vi "Main2.vi"() -> ()   [LabVIEW 2024]
uses:
  Global 1.vi
  Control 1.ctl
panel:
  in  "Array 3":string[][](array[string])=[["dsfds", "-797", "-798", "-1.00", "No Alarm", "<", "12"]]
  out "Waveform Graph":dbl[][](graph)
  out "Array 2":string[][](array[string])
  out "# Of Curr Paramters":dbl
  out "# Of total Paramters":dbl
  in  "Print Button":bool
  out "Current Running Test":string
  in  "Rate of change":T1(array[cluster])
  out "Numeric":dbl
  out "error out":errorcluster
  out "Time Elapsed?":bool=TRUE
  out "Paused?":bool
  in  "error in (no error)":errorcluster
  in  "Select Time":enum16{"Reset", "Start", "Pause", "Unpause"}(ring)=enum."Start"
  in  "Array 4":T2(array[cluster])
  out "Table Control":string[][](table)
  # "Timer"
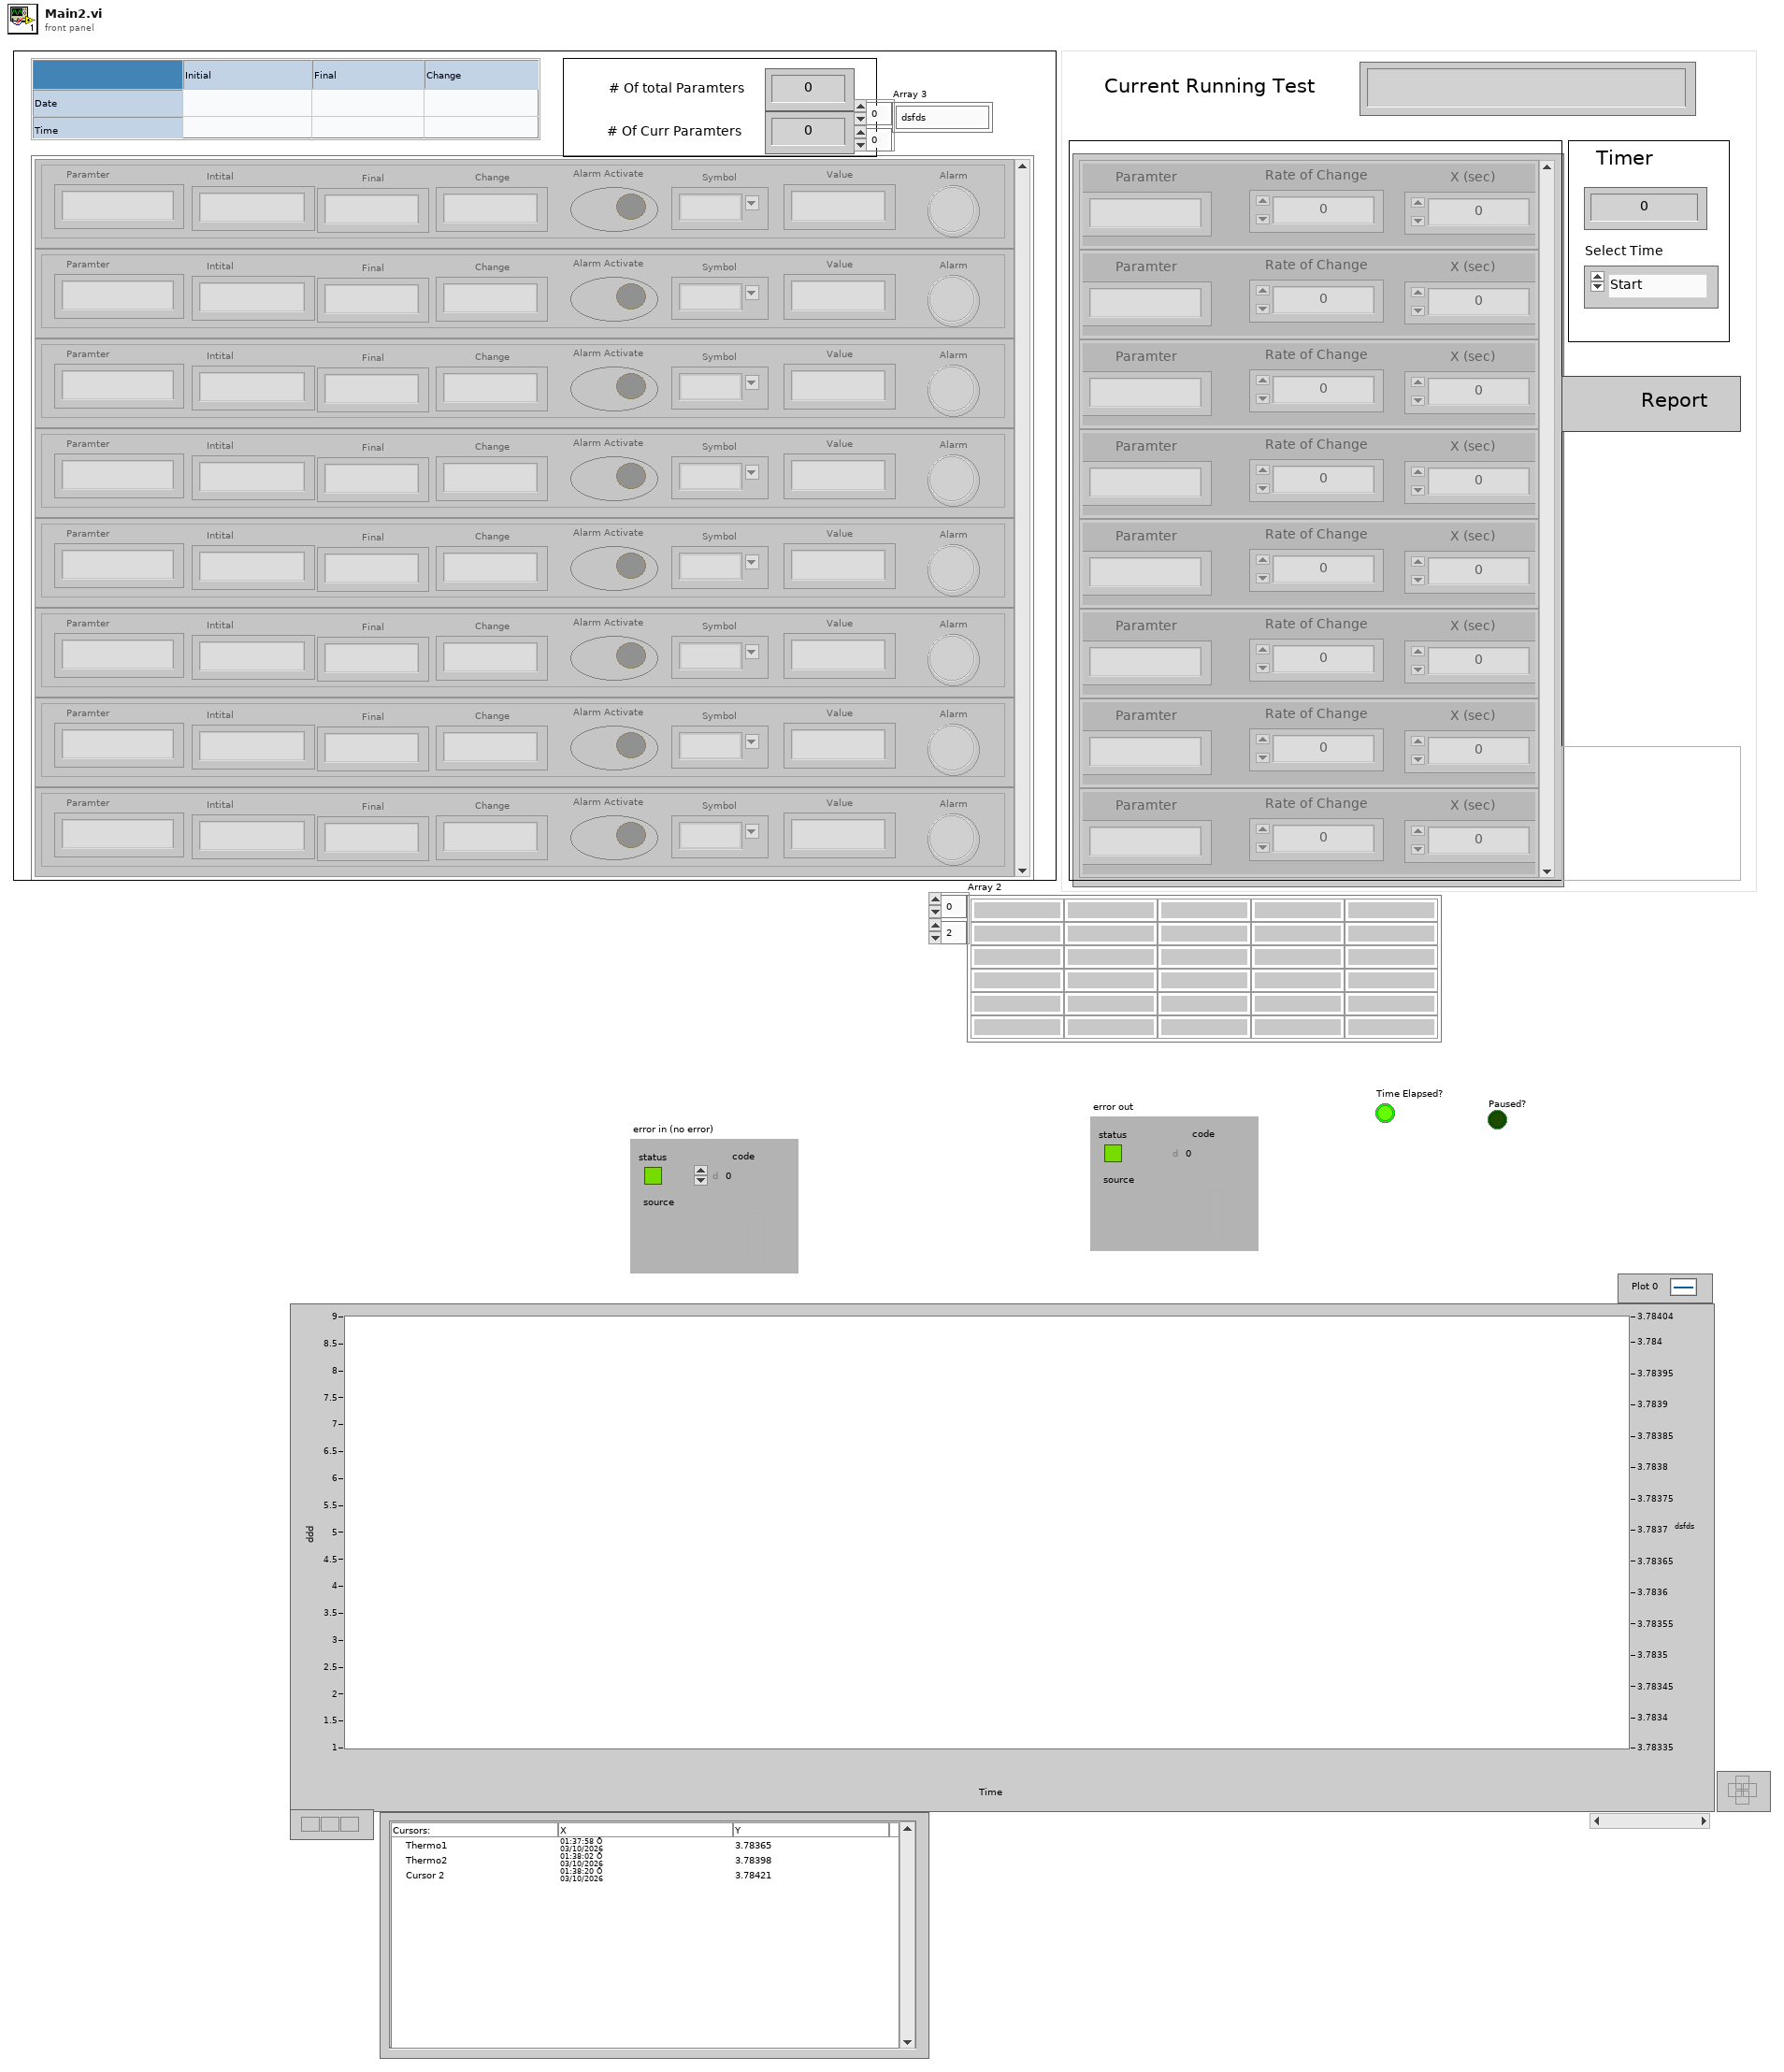
[diagram p1: front panel]
types:
  T1 = cluster{"Paramter":string, "Rate of Change":dbl, "X (sec)":dbl}[]
  T2 = cluster{"Paramter":string, "Intital ":string, "Final":string, "Change":string, "Alarm Activate ":bool, "Symbol":string, "Value":string, "Alarm":bool}[]
  T3 = cluster{"Paramter":string, "Rate of Change":dbl, "X (min)":dbl}[]
  T4 = cluster{"Paramter":string, "Rate of Change":dbl, "X Min":string}[]
  T5 = typedef "Control 1.ctl" = enum16{"Start", "Initialize"}
  T6 = cluster{"Paramter":string, "Rate of Change":dbl, "X (min)":dbl}
  T7 = cluster{"Paramter":string, "Intital ":string, "Final":string, "Change":string, "Alarm Activate ":bool, "Symbol":string, "Value":string, "Alarm":bool}
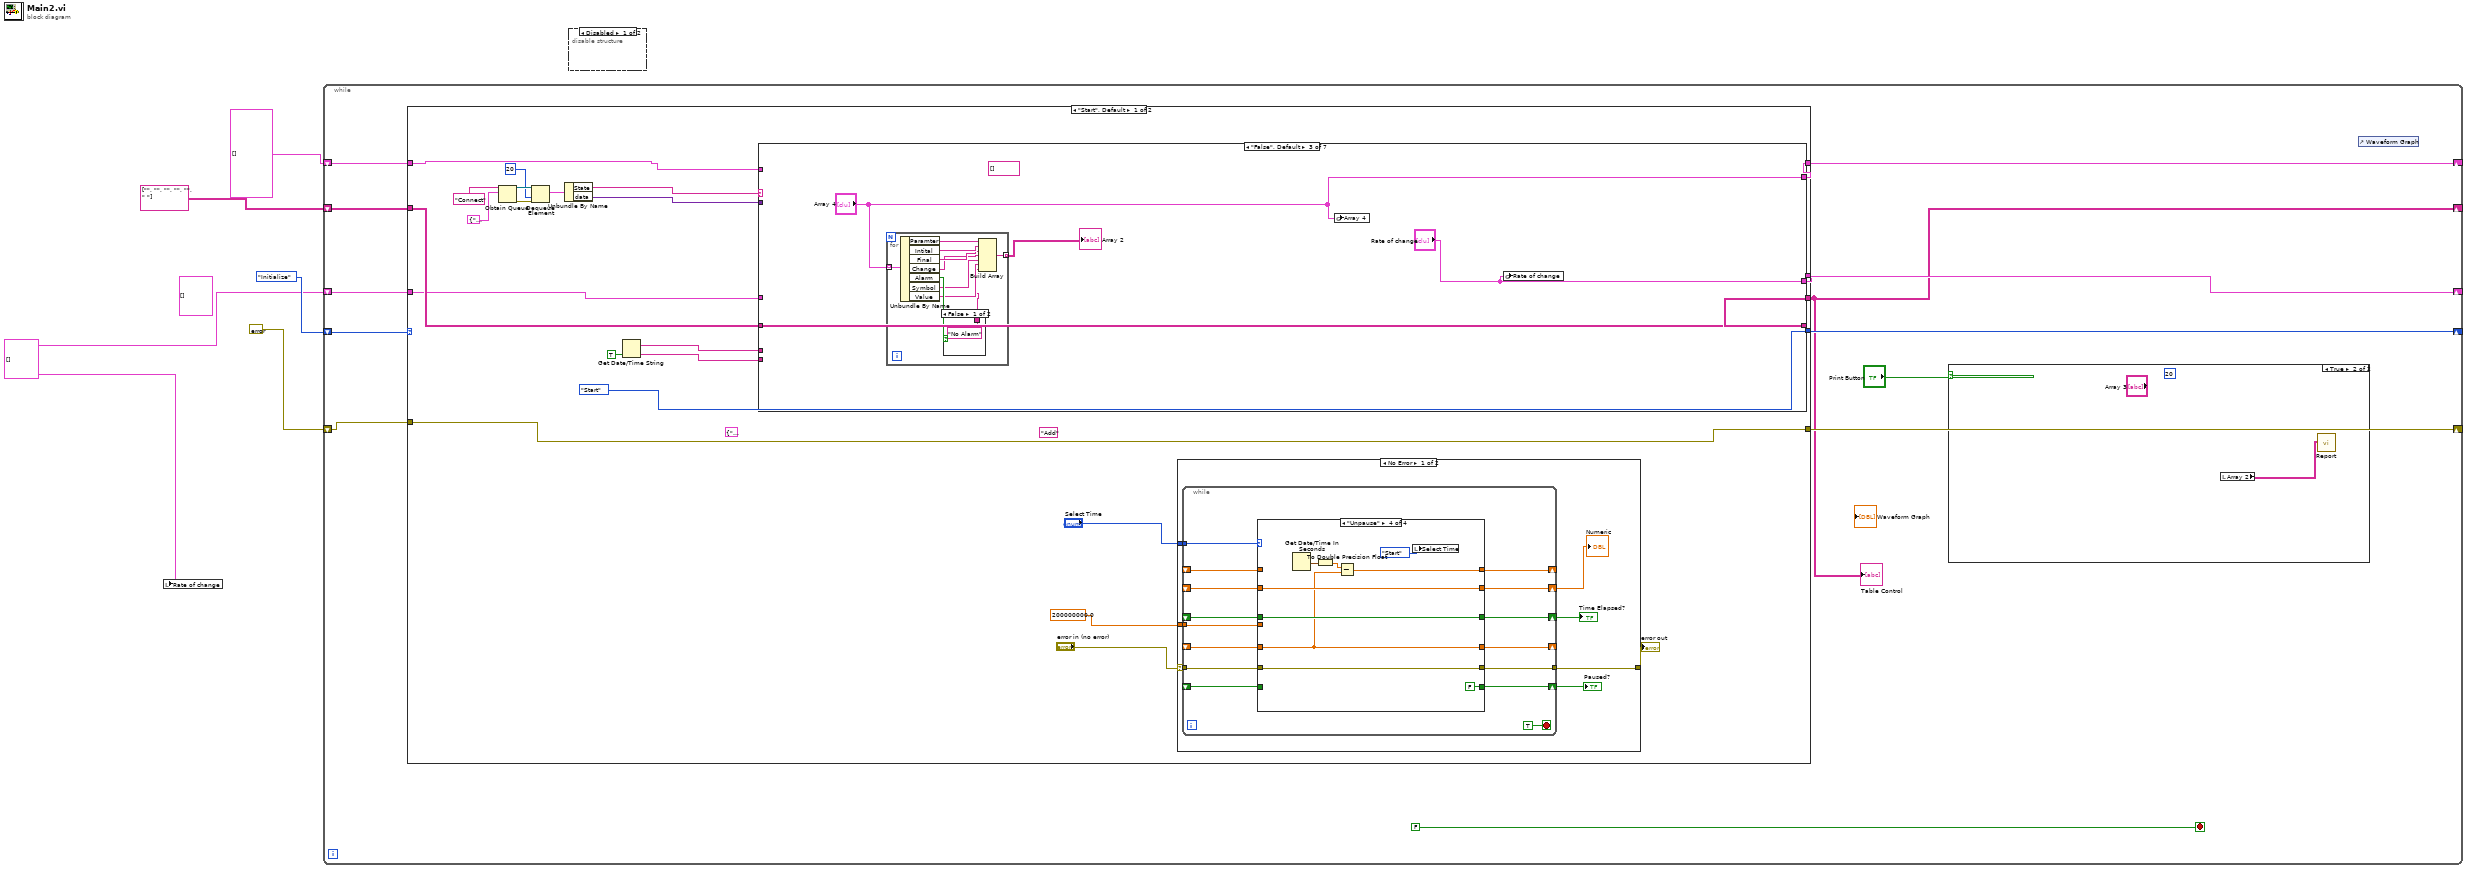
[diagram p0: block diagram]
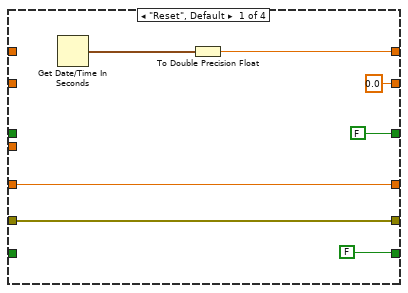
[diagram p4: hidden frame]
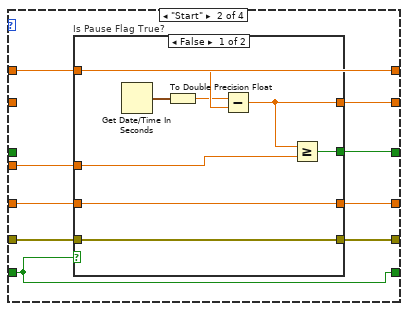
[diagram p5: hidden frame]
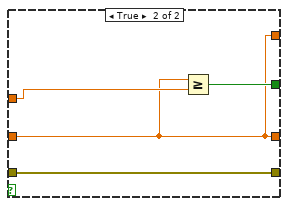
[diagram p6: hidden frame]
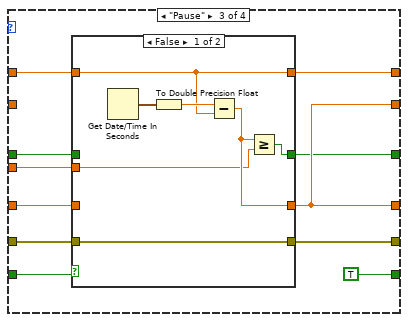
[diagram p7: hidden frame]
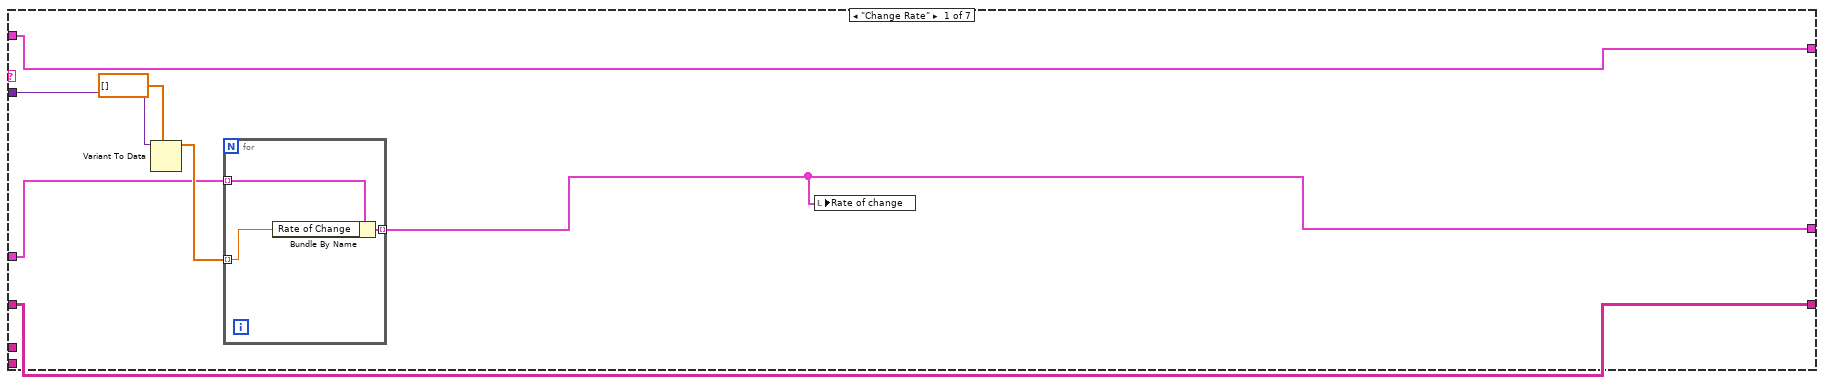
[diagram p10: hidden frame]
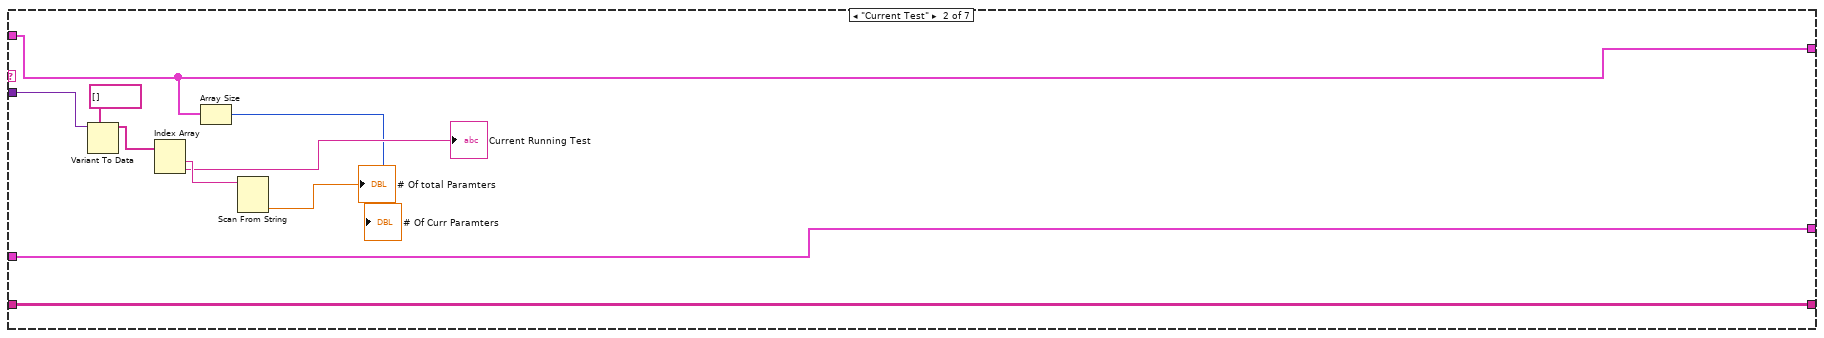
[diagram p11: hidden frame]
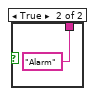
[diagram p12: hidden frame]
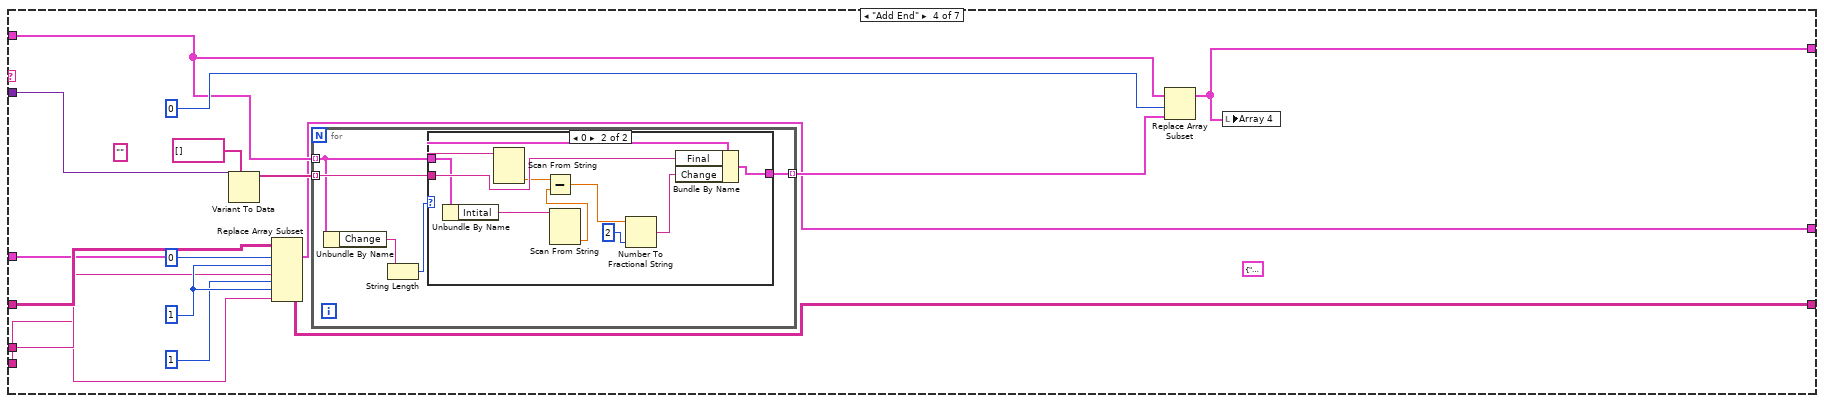
[diagram p13: hidden frame]
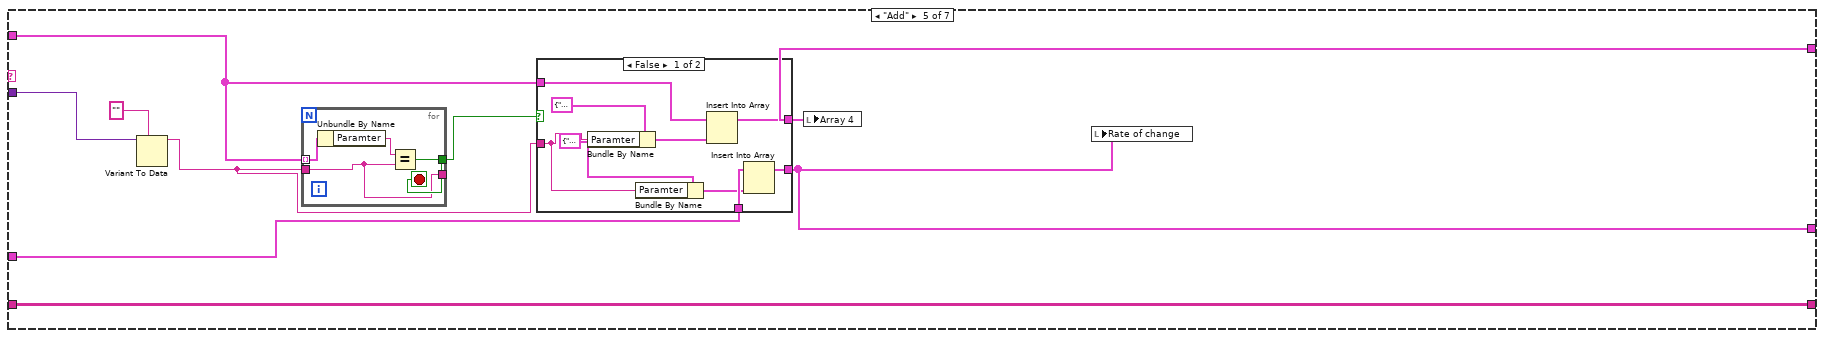
[diagram p15: hidden frame]
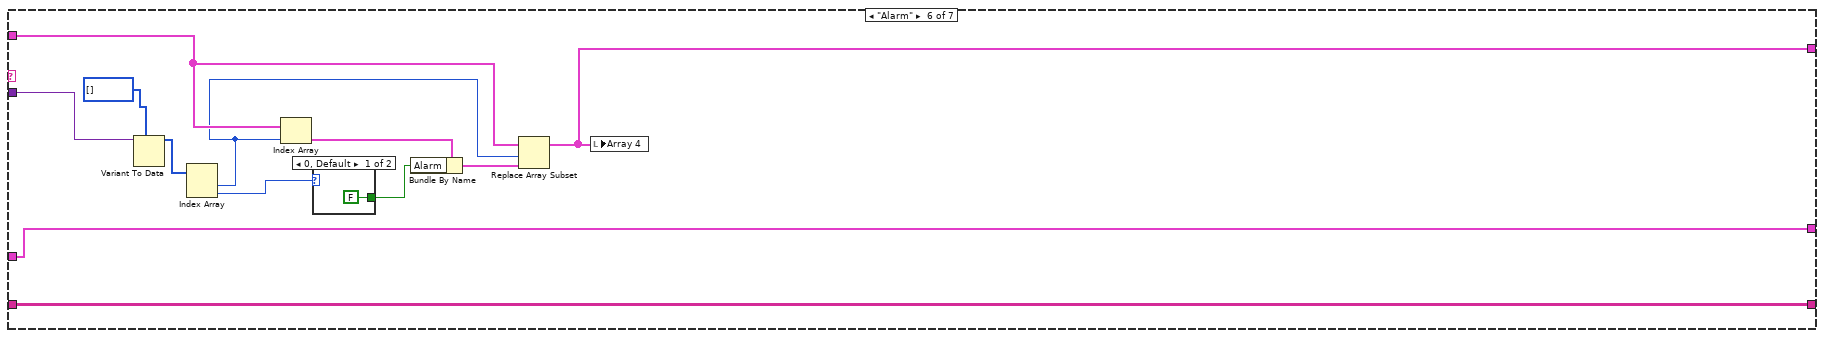
[diagram p17: hidden frame]
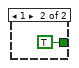
[diagram p18: hidden frame]
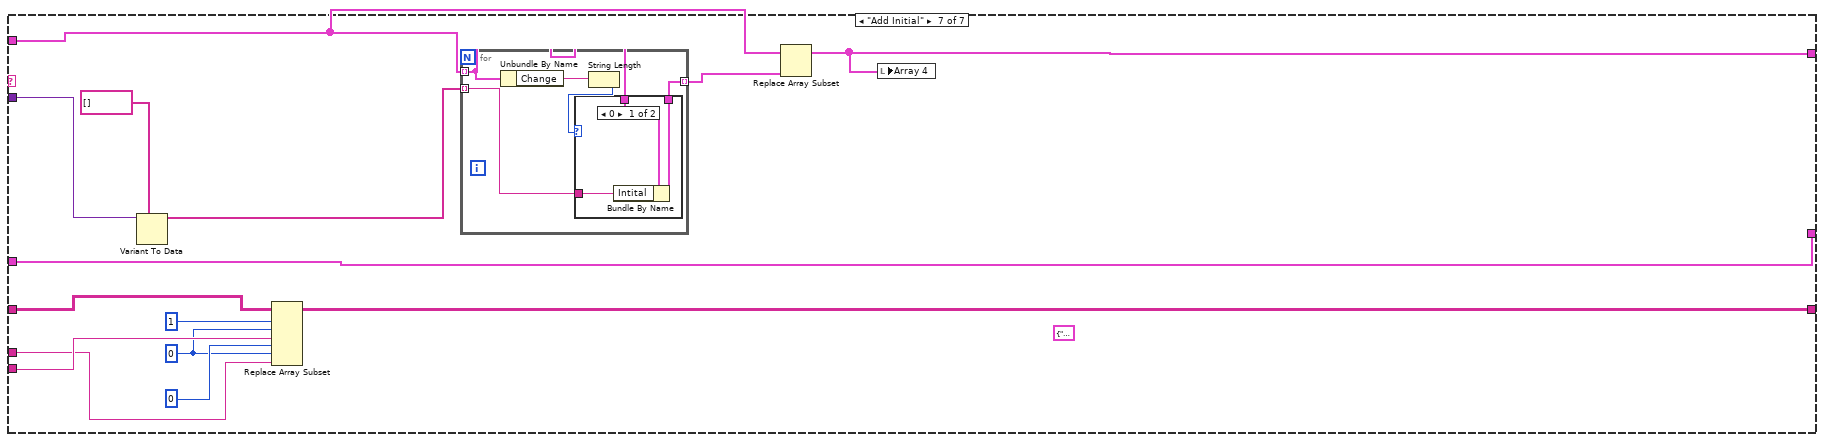
[diagram p19: hidden frame]
diagram:
  w1 = T3 []
  (unwired) T4 [] ("Array")
  n1 = local write "Rate of change"(w1) -> ()
  n2 = while {
    shift-right: [w15] -> _
    shift-left: Control_1."Initialize" -> [w16]
    shift-right: [w11] -> _
    shift-left: T2 [] ("Array 4") -> [w10]
    shift-right: [w13] -> _
    shift-left: errorcluster {"status"=FALSE, "code"=0, "source"=""} ("error constant") -> [w14]
    shift-right: [w7] -> _
    shift-left: string[][] [["", "", ""], ["", "", " "]] ("Table Control") -> [w12]
    shift-right: [w8] -> _
    shift-left: w1 -> [w9]
    stop <- FALSE stop-if-true
    n3 = case shown="\"Start\", Default" w16 {
      tunnel: [Control_1."Start" Control_1."Start"] -> w15
      tunnel: w10 -> [w19 w259]
      tunnel: [w33 w259] -> w11
      tunnel: w14 -> [w32 w257]
      tunnel: [w32 w256] -> w13
      tunnel: w12 -> [w30 w255]
      tunnel: [w27 w255] -> w7
      tunnel: w9 -> [w21 w254]
      tunnel: [w20 w254] -> w8
      frame "Start", Default {
        (unwired) "Add" ("State")
        (unwired) cluster{"State":string, "data":variant} {"State"="", "data"=variant}
        n4 = Obtain Queue(name (unnamed)="Connect", element data type=cluster{"State":string, "data":variant} {"State"="", "data"=variant}) -> (queue out=w39:refnum<queue>, error out=w40:errorcluster)  [unwired: 3 in, 1 out]
        n5 = Dequeue Element(queue=w39, timeout in ms (-1)=20, error in (no error)=w40) -> (element=w36:cluster{"State":string, "data":variant})  [unwired: 3 out]
        n6 = Unbundle By Name(w36) -> ("State"=w35:string, "data"=w34:variant)
        n7 = Get Date/Time String(want seconds? (F)=TRUE) -> (date string=w26:string, time string=w28:string)  [unwired: 2 in]
        n8 = case shown="\"False\", Default" w35 {
          tunnel: w34 -> [w130 w143 _ w164 w198 w225 w240]
          tunnel: w19 -> [w127 w135 _ w163 w194 w223 w230]
          tunnel: [w127 w135 "Array 4" w166 w196 w220 w241] -> w33
          tunnel: w30 -> [w126 w141 w147 w171 w195 w221 w239]
          tunnel: [w126 w141 w147 w170 w195 w221 w236] -> w27
          tunnel: w28 -> [_ _ _ w168 _ _ w237]
          tunnel: w26 -> [_ _ _ w169 _ _ w233]
          tunnel: w21 -> [w125 w142 _ w160 w192 w219 w229]
          tunnel: [w124 w142 "Rate of change" w160 w191 w219 w229] -> w20
          frame "Change Rate" {
            n9 = Variant To Data(type=dbl[] [], Variant=w130) -> (data=w128:dbl[])  [unwired: 1 in, 1 out]
            n10 = for {
              tunnel: w128 -> [w133] mode=indexing
              tunnel: [w132] -> w124 mode=indexing
              tunnel: w125 -> [w131] mode=indexing
              n11 = Bundle By Name(cluster=w131, "Rate of Change"=w133) -> (w132:T6)
            }
            n12 = local write "Rate of change"(w124) -> ()
          }
          frame "Current Test" {
            n13 = Variant To Data(type=string[] [], Variant=w143) -> (data=w139:string[])  [unwired: 1 in, 1 out]
            n14 = Index Array(array=w139) -> (element #1=w137:string, element #2=→"Current Running Test":string)  [unwired: 2 in]
            n15 = Array Size(array=w135) -> (size(s)=→"# Of Curr Paramters":i32)
            n16 = Scan From String(input string=w137) -> (output 1=→"# Of total Paramters":dbl)  [unwired: 4 in, 3 out]
          }
          frame "False", Default {
            (unwired) string[] []
            n17 = for {
              tunnel: "Array 4" -> [w157] mode=indexing
              tunnel: [w151] -> w144 mode=indexing
              n18 = Unbundle By Name(w157) -> ("Paramter"=w155:string, "Intital"=w154:string, "Final"=w153:string, "Change"=w152:string, "Alarm"=w156:bool, "Symbol"=w150:string, "Value"=w149:string)
              n19 = case shown="False" w156 {
                tunnel: ["No Alarm" "Alarm"] -> w148
                frame False {
                }
                frame True {
                }
              }
              n20 = Build Array(w155, w154, w153, w152, w150, w149, w148) -> (w151:string[])
            }
            "Array 2" <- w144
            n21 = global write "Global 1.vi" "Array 4"("Array 4") -> ()
            n22 = global write "Global 1.vi" "Rate of change"("Rate of change") -> ()
          }
          frame "Add End" {
            w173 = 1 ("disabled index (col)")
            (unwired) ""
            (unwired) T7 {"Paramter"="", "Intital "="", "Final"="", "Change"="", "Alarm Activate "=FALSE, "Symbol"="", "Value"="", "Alarm"=FALSE} ("new element/subarray")
            n23 = Variant To Data(type=string[] [], Variant=w164) -> (data=w162:string[])  [unwired: 1 in, 1 out]
            n24 = Replace Array Subset(array=w171, new element #1=w169, index (row) #1=0 ("index (row)"), index (col) #1=w173, new element #2=w168, index (row) #2=1 ("index (row)"), index (col) #2=w173) -> (w170:string[][])
            n25 = for {
              tunnel: w163 -> [w177] mode=indexing
              tunnel: w162 -> [w178] mode=indexing
              tunnel: [w179] -> w161 mode=indexing
              n26 = Unbundle By Name(w177) -> ("Change"=w176:string)
              n27 = String Length(string=w176) -> (length=w175:i32)
              n28 = case shown="0" w175 {
                tunnel: [w180 w189] -> w179
                tunnel: w178 -> [_ w188]
                tunnel: w177 -> [w180 w181]
                frame 1, Default {
                }
                frame 0 {
                  n29 = Unbundle By Name(w181) -> ("Intital"=w182:string)
                  n30 = Scan From String(input string=w188) -> (output 1=w186:dbl)  [unwired: 4 in, 3 out]
                  n31 = Scan From String(input string=w182) -> (output 1=w187:dbl)  [unwired: 4 in, 3 out]
                  n32 = Subtract(x=w186, y=w187) -> (x-y=w184:dbl)
                  n33 = Number To Fractional String(number=w184, precision (6)=i16 2) -> (F-format string=w183:string)  [unwired: 2 in]
                  n34 = Bundle By Name(cluster=w181, "Final"=w188, "Change"=w183) -> (w189:T7)
                }
              }
            }
            n35 = Replace Array Subset(array=w163, new element=w161, index=0) -> (w166:T2)
            n36 = local write "Array 4"(w166) -> ()
          }
          frame "Add" {
            n37 = Variant To Data(type="", Variant=w198) -> (data=w190:string)  [unwired: 1 in, 1 out]
            n38 = for {
              tunnel: w194 -> [w213] mode=indexing
              tunnel: w190 -> [w210]
              tunnel: [w211] -> w193
              tunnel: [w210] -> _
              stop <- w211 stop-if-true
              n39 = Unbundle By Name(w213) -> ("Paramter"=w212:string)
              n40 = Equal?(x=w212, y=w210) -> (x = y?=w211:bool)
            }
            n41 = case shown="False" w193 {
              tunnel: [w205 w209] -> w196
              tunnel: w194 -> [w204 w209]
              tunnel: w190 -> [w203 _]
              tunnel: w192 -> [w201 w208]
              tunnel: [w199 w208] -> w191
              frame False {
                n42 = Bundle By Name(cluster=T7 {"Paramter"="", "Intital "="", "Final"="", "Change"="", "Alarm Activate "=FALSE, "Symbol"="", "Value"="", "Alarm"=FALSE} ("new element/subarray"), "Paramter"=w203) -> (w206:T7)
                n43 = Bundle By Name(cluster=T6 {"Paramter"="vvc", "Rate of Change"=0.0, "X (min)"=0.0} ("Rate Of Change"), "Paramter"=w203) -> (w200:T6)
                n44 = Insert Into Array(array=w204, new element=w206) -> (w205:T2)  [unwired: 1 in]
                n45 = Insert Into Array(array=w201, new element=w200) -> (w199:T3)  [unwired: 1 in]
              }
              frame True {
              }
            }
            n46 = local write "Array 4"(w196) -> ()
            n47 = local write "Rate of change"(w191) -> ()
          }
          frame "Alarm" {
            n48 = Variant To Data(type=i32[] [], Variant=w225) -> (data=w217:i32[])  [unwired: 1 in, 1 out]
            n49 = Index Array(array=w217) -> (element #1=w216:i32, element #2=w214:i32)  [unwired: 2 in]
            n50 = Index Array(array=w223, index=w216) -> (element=w224:T7)
            n51 = case shown="0, Default" w214 {
              tunnel: [FALSE ("Alarm") TRUE ("Alarm")] -> w215
              frame 0, Default {
              }
              frame 1 {
              }
            }
            n52 = Bundle By Name(cluster=w224, "Alarm"=w215) -> (w222:T7)
            n53 = Replace Array Subset(array=w223, new element=w222, index=w216) -> (w220:T2)
            n54 = local write "Array 4"(w220) -> ()
          }
          frame "Add Initial" {
            w234 = 0 ("disabled index (col)")
            (unwired) T7 {"Paramter"="", "Intital "="", "Final"="", "Change"="", "Alarm Activate "=FALSE, "Symbol"="", "Value"="", "Alarm"=FALSE} ("new element/subarray")
            n55 = Variant To Data(type=string[] [], Variant=w240) -> (data=w228:string[])  [unwired: 1 in, 1 out]
            n56 = Replace Array Subset(array=w239, new element #1=w237, index (row) #1=1 ("index (row)"), index (col) #1=w234, new element #2=w233, index (row) #2=0 ("index (row)"), index (col) #2=w234) -> (w236:string[][])
            n57 = for {
              tunnel: w228 -> [w245] mode=indexing
              tunnel: [w246] -> w231 mode=indexing
              tunnel: w230 -> [w243] mode=indexing
              n58 = Unbundle By Name(w243) -> ("Change"=w244:string)
              n59 = String Length(string=w244) -> (length=w242:i32)
              n60 = case shown="0" w242 {
                tunnel: [w249 w250] -> w246
                tunnel: w245 -> [w248 _]
                tunnel: w243 -> [w247 w250]
                frame 0 {
                  n61 = Bundle By Name(cluster=w247, "Intital"=w248) -> (w249:T7)
                }
                frame 1, Default {
                }
              }
            }
            n62 = Replace Array Subset(array=w230, new element=w231) -> (w241:T2)  [unwired: 1 in]
            n63 = local write "Array 4"(w241) -> ()
          }
        }
        n64 = case shown="No Error" "error in (no error)" {
          selector: "error in (no error)" -> [w47 w123]
          tunnel: [w48 w123] -> w24
          tunnel: "Select Time" -> [w46 _]
          tunnel: 200000000.0 ("Target Time") -> [w44 _]
          frame No Error {
            n65 = while {
              tunnel: [w62] -> w48
              tunnel: w47 -> [w61]
              tunnel: w46 -> [w60]
              shift-right: [w59] -> _
              shift-left: _ -> [w58]
              tunnel: w44 -> [w55]
              shift-right: [w54] -> _
              shift-left: _ -> [w51]
              shift-right: [w53] -> w43
              shift-left: _ -> [w52]
              shift-right: [w56] -> w45
              shift-left: _ -> [w50]
              shift-right: [w57] -> w42
              shift-left: _ -> [w49]
              stop <- TRUE stop-if-true
              n66 = case shown="\"Unpause\"" w60 {
                tunnel: [w70 w72 w99 w121] -> w62
                tunnel: w61 -> [w70 w71 w98 w121]
                tunnel: [w66 w79 w95 w118] -> w59
                tunnel: w58 -> [_ w79 w102 _]
                tunnel: [0.0 w78 w100 w117] -> w57
                tunnel: [FALSE w76 w94 w116] -> w56
                tunnel: w55 -> [_ w77 w92 _]
                tunnel: [w64 w73 w100 w115] -> w54
                tunnel: [FALSE w75 TRUE FALSE] -> w53
                tunnel: w52 -> [_ w75 w97 _]
                tunnel: w51 -> [w64 w74 w96 w115]
                tunnel: w50 -> [_ _ w93 w116]
                tunnel: w49 -> [_ _ _ w117]
                frame "Reset", Default {
                  n67 = Get Date/Time In Seconds() -> (seconds since 1Jan1904=w67:timestamp)
                  n68 = To Double Precision Float(number=w67) -> (double precision float=w66:dbl)
                }
                frame "Start" {
                  n69 = case "Is Pause Flag True?" shown="False" w75 {
                    tunnel: w79 -> [w87 _]
                    tunnel: [w80 w89] -> w78
                    tunnel: w77 -> [w86 w90]
                    tunnel: [w85 w91] -> w76
                    tunnel: w74 -> [w82 w89]
                    tunnel: [w82 w89] -> w73
                    tunnel: [w81 w88] -> w72
                    tunnel: w71 -> [w81 w88]
                    frame False {
                      n70 = Get Date/Time In Seconds() -> (seconds since 1Jan1904=w84:timestamp)
                      n71 = To Double Precision Float(number=w84) -> (double precision float=w83:dbl)
                      n72 = Subtract(x=w83, y=w87) -> (x-y=w80:dbl)
                      n73 = Greater Or Equal?(x=w80, y=w86) -> (x >= y?=w85:bool)
                    }
                    frame True {
                      n74 = Greater Or Equal?(x=w89, y=w90) -> (x >= y?=w91:bool)
                    }
                  }
                }
                frame "Pause" {
                  n75 = case shown="False" w97 {
                    tunnel: w102 -> [w106 w112]
                    tunnel: [w105 w113] -> w100
                    tunnel: [w107 w111] -> w99
                    tunnel: w98 -> [w107 w111]
                    tunnel: w96 -> [_ w113]
                    tunnel: [w106 w112] -> w95
                    tunnel: [w103 w110] -> w94
                    tunnel: w93 -> [_ w110]
                    tunnel: w92 -> [w104 _]
                    frame False {
                      n76 = Get Date/Time In Seconds() -> (seconds since 1Jan1904=w108:timestamp)
                      n77 = To Double Precision Float(number=w108) -> (double precision float=w109:dbl)
                      n78 = Subtract(x=w109, y=w106) -> (x-y=w105:dbl)
                      n79 = Greater Or Equal?(x=w105, y=w104) -> (x >= y?=w103:bool)
                    }
                    frame True {
                    }
                  }
                }
                frame "Unpause" {
                  n80 = Get Date/Time In Seconds() -> (seconds since 1Jan1904=w119:timestamp)
                  n81 = To Double Precision Float(number=w119) -> (double precision float=w120:dbl)
                  n82 = Subtract(x=w120, y=w115) -> (x-y=w118:dbl)
                  n83 = local write "Select Time"(enum16{"Reset", "Start", "Pause", "Unpause"}."Start" ("Select Time")) -> ()
                }
              }
            }
            "Time Elapsed?" <- w45
            "Paused?" <- w43
            "Numeric" <- w42
          }
          frame Error {
          }
        }
        "error out" <- w24
      }
      frame "Initialize" {
        w258 = T2 [] ("Array 4")
        n84 = global write "Global 1.vi" "Array 4"(w258) -> ()
        n85 = property on="Array 4" class="Arr (strict)"(error in=w257, "Value"=w258) -> (error out=w256:errorcluster)  [unwired: 1 in, 1 out]
        n86 = property on="Current Running Test" class="Str"("Value"="" ("Current Running Test")) -> ()  [unwired: 2 in, 2 out]
        n87 = local write "Select Time"(enum16{"Reset", "Start", "Pause", "Unpause"}."Reset" ("Select Time")) -> ()
        n88 = property on="# Of total Paramters" class="DigNum (strict)"("Value"=0.0 ("# Of total Paramters")) -> ()  [unwired: 2 in, 2 out]
      }
    }
    "Table Control" <- w7
    n89 = case shown="True" "Print Button" {
      frame False {
      }
      frame True {
        (unwired) 20 ("timeout in ms (-1)")
        n90 = local read "Array 2"() -> (w18:string[][])
        n91 = call "Report.vi"("Array 2"=w18) -> ()  [unwired: 11 in]
      }
    }
    n92 = control-ref of="Waveform Graph"() -> ()  [unwired: 1 out]
  }
  n93 = disable-structure shown="Disabled" {
    frame Disabled {
    }
    frame Enabled {
    }
  }
